vi "filter_edge_detect_3.vi"(0 "image in":T1, 1 "mid Lane Options":T2 {"Edge Polarity" items=["All Edges", "Rising Edges", "Falling Edges"]; "Minimum Edge Strength" format="%.2f"; "Width" step=2; "Kernel Size" step=2}, 2 "right Lane Descriptor":T4, 3 "left Lane Descriptor":T4, 4 "mid Lane Descriptor":T4, 5 "error in (no error)":errorcluster, 6 "Color Plane":i32(ring)=1 items=["Red", "Green", "Blue", "Hue", "Saturation", "Luminance", "Value", "Intensity"], 7 "Lane_center":dbl, 8 "Lane Process":T6(ring)=enum."Get First + Last Edge", 9 "Right Process":T6(ring)=enum."Get First + Last Edge", 10 "Left Options":T2 {"Edge Polarity" items=["All Edges", "Rising Edges", "Falling Edges"]; "Minimum Edge Strength" format="%.2f"; "Width" step=2; "Kernel Size" step=2}, 11 "Right Options":T2 {"Edge Polarity" items=["All Edges", "Rising Edges", "Falling Edges"]; "Minimum Edge Strength" format="%.2f"; "Width" step=2; "Kernel Size" step=2}, 12 "Left Process":T6(ring)=enum."Get First + Last Edge") -> (13 "right_edge_location":cluster{"X":sgl, "Y":sgl}[](array[cluster]), 14 "image out":T1, 15 "Mid Edge Information":T5[](array[typedef]) {"Distance (Real-World)" format="%.2f"; "Location (Real-World)"."Y" format="%.2g"; "Location (Real-World)"."X" format="%.2f"; "Noise" format="%.2f"; "Location (Pixel)"."Y" format="%.2g"; "Location (Pixel)"."X" format="%.2f"; "Strength" format="%.2f"; "Distance (Pixel)" format="%.2f"}, 16 "Left Edge Information":T5[](array[typedef]) {"Distance (Real-World)" format="%.2f"; "Location (Real-World)"."Y" format="%.2g"; "Location (Real-World)"."X" format="%.2f"; "Noise" format="%.2f"; "Location (Pixel)"."Y" format="%.2g"; "Location (Pixel)"."X" format="%.2f"; "Strength" format="%.2f"; "Distance (Pixel)" format="%.2f"}, 17 "Right Edge Information":T5[](array[typedef]) {"Distance (Real-World)" format="%.2f"; "Location (Real-World)"."Y" format="%.2g"; "Location (Real-World)"."X" format="%.2f"; "Noise" format="%.2f"; "Location (Pixel)"."Y" format="%.2g"; "Location (Pixel)"."X" format="%.2f"; "Strength" format="%.2f"; "Distance (Pixel)" format="%.2f"}, 18 "mid_edge_location":cluster{"X":sgl, "Y":sgl}[](array[cluster]), 19 "left_edge_location":cluster{"X":sgl, "Y":sgl}[](array[cluster]))   [LabVIEW 2024]
uses:
  <vilib>/vision/Measure.llb/Edge New.ctl
  <vilib>/vision/Image Controls.llb/IMAQ Image.ctl
  <vilib>/vision/Measure.llb/Edge Options.ctl
  <vilib>/vision/Measure.llb/Edge Polarity.ctl
  <vilib>/vision/NI_Vision_Development_Module.lvlib
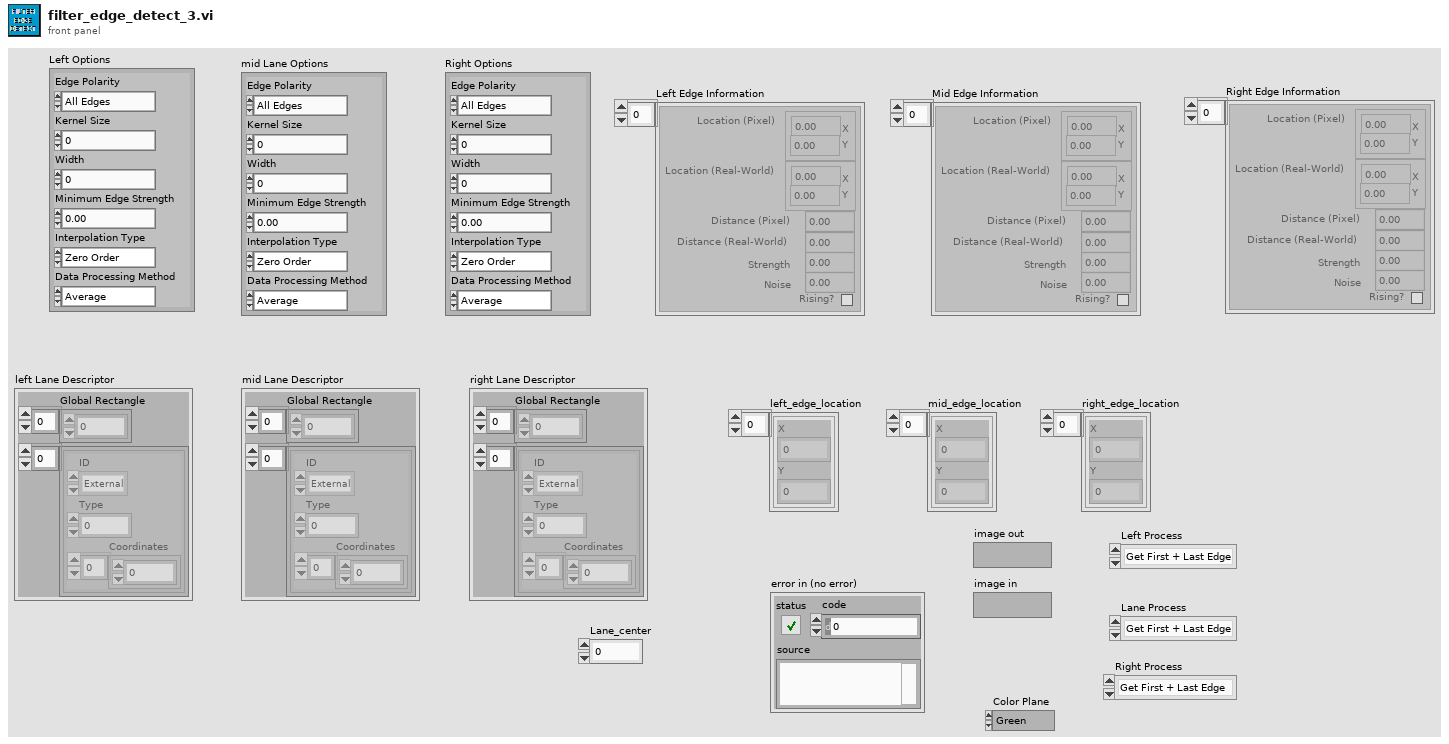
[diagram p1: front panel]
types:
  T1 = typedef "IMAQ Image.ctl" = refnum<image>
  T2 = typedef "Edge Options.ctl" = cluster{"Edge Polarity":T3, "Kernel Size":u32, "Width":u32, "Minimum Edge Strength":sgl, "Interpolation Type":enum32{"Zero Order", "Bilinear", "Quadratic", "Cubic", "Bilinear Fixed"}, "Data Processing Method":enum32{"Average", "Median"}}
  T3 = typedef "Edge Polarity.ctl" = u32
  T4 = cluster{"Global Rectangle":i32[], cluster{"ID":enum32{"External", "Internal"}, "Type":u32, "Coordinates":i32[]}[]}
  T5 = typedef "Edge New.ctl" = cluster{"Location (Pixel)":cluster{"X":sgl, "Y":sgl}, "Location (Real-World)":cluster{"X":sgl, "Y":sgl}, "Distance (Pixel)":dbl, "Distance (Real-World)":dbl, "Strength":dbl, "Noise":dbl, "Rising?":bool}
  T6 = enum16{"Get First Edge", "Get First + Last Edge", "Get All Edges", "Get Best Edge"}
  T7 = cluster{"ID":enum32{"External", "Internal"}, "Type":u32, "Coordinates":i32[]}[]
  T8 = cluster{"ID":enum32{"External", "Internal"}, "Type":u32, "Coordinates":i32[]}
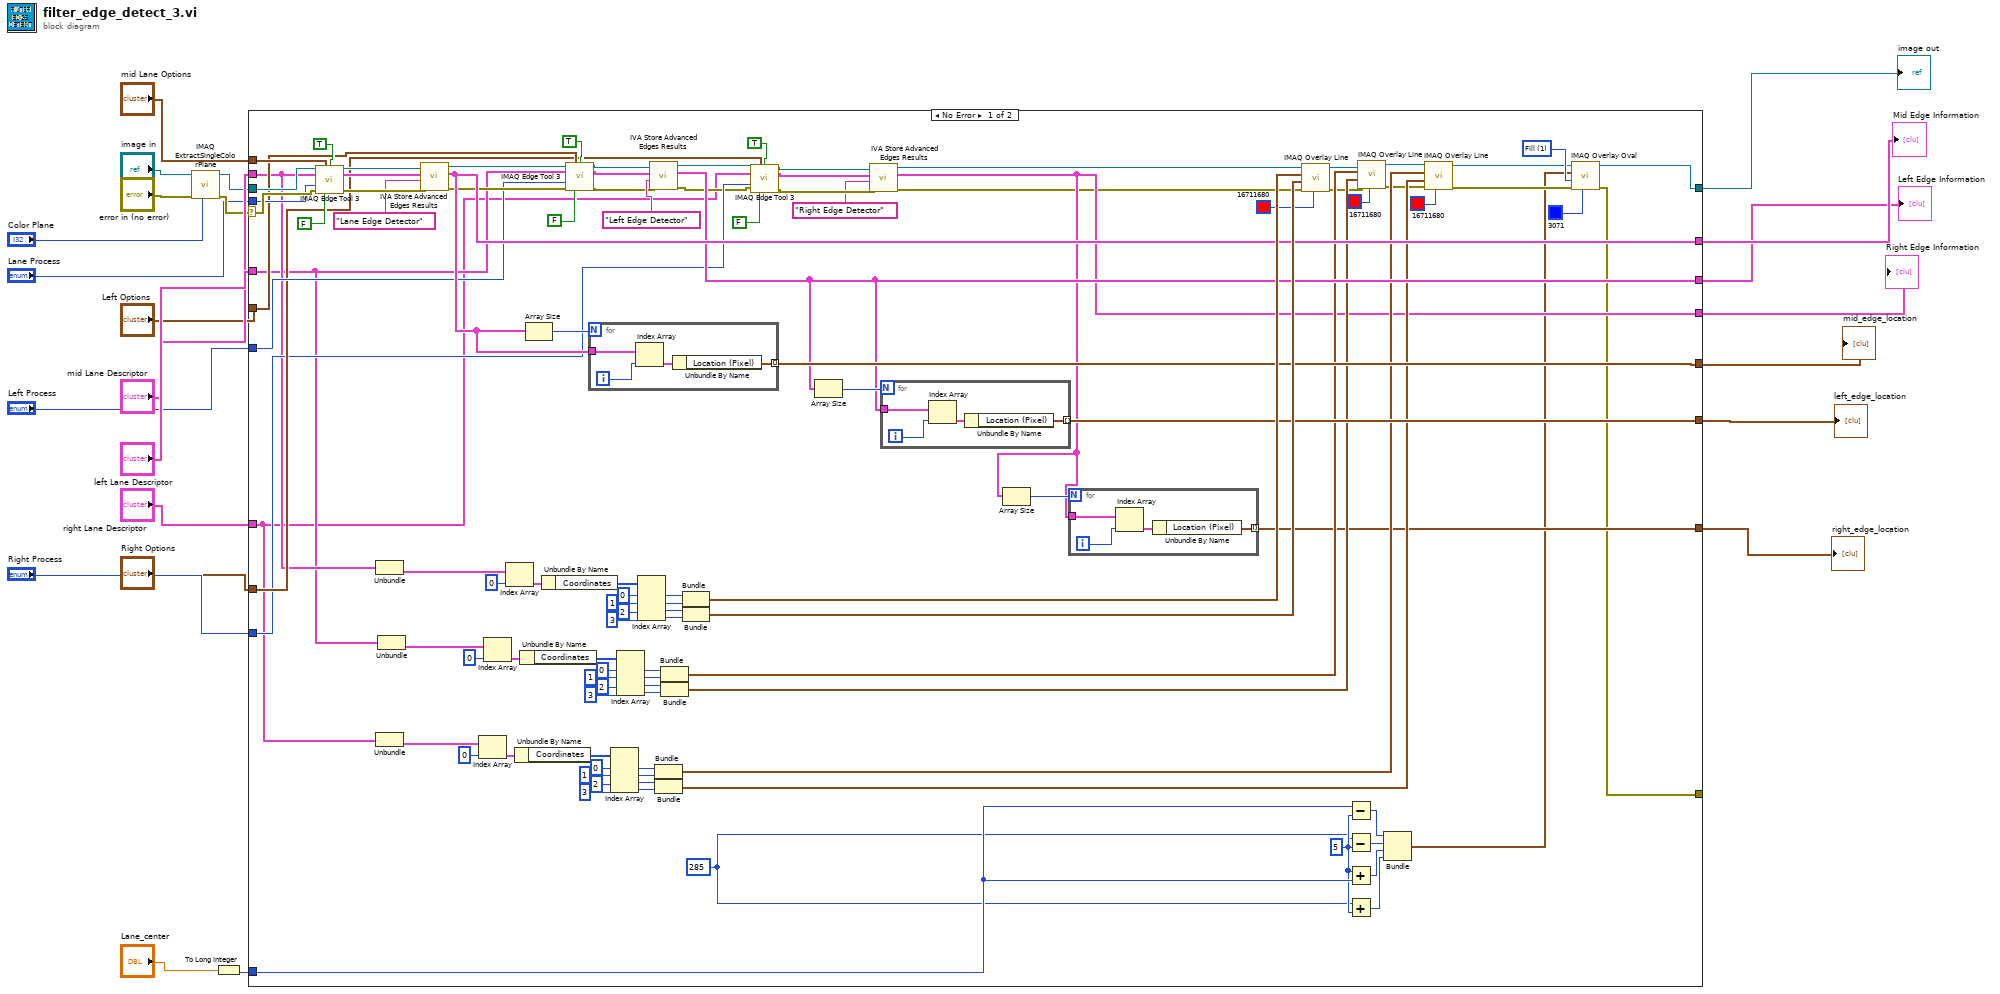
[diagram p0: block diagram]
diagram:
  n1 = call "IMAQ ExtractSingleColorPlane"("Color Plane"="Color Plane", "error in (no error)"="error in (no error)", "Image Src"="image in") -> ("error out"=w4:errorcluster, "Image Dst Out"=w5:T1)  [unwired: 1 in, 6 out]
  n2 = To Long Integer(number="Lane_center") -> (32bit integer=w22:i32)
  n3 = case shown="No Error" w4 {
    selector: w4 -> [w130 w144]
    tunnel: [w33 w144] -> _
    tunnel: w5 -> [w129 w143]
    tunnel: "mid Lane Descriptor" -> [w44 _]
    tunnel: "Lane Process" -> [w128 _]
    tunnel: "mid Lane Options" -> [w126 _]
    tunnel: [w98 _] -> w17
    tunnel: "left Lane Descriptor" -> [w41 _]
    tunnel: "Left Options" -> [w97 _]
    tunnel: "Left Process" -> [w95 _]
    tunnel: [w94 _] -> w19
    tunnel: [w74 _] -> w16
    tunnel: [w75 _] -> w20
    tunnel: "right Lane Descriptor" -> [w39 _]
    tunnel: "Right Options" -> [w69 _]
    tunnel: "Right Process" -> [w68 _]
    tunnel: [w51 _] -> w18
    tunnel: [w35 w143] -> w12
    tunnel: [w38 _] -> w21
    tunnel: w22 -> [w30 _]
    frame No Error {
      w24 = 285 ("y")
      w27 = 5 ("y")
      w37 = u32 1 items=["Frame", "Fill"] ("Drawing Mode (Frame)")
      n4 = call "IMAQ Edge Tool 3"("Image"=w129, "Edge Options"=w126, "Optimized Mode"=TRUE, "ROI Descriptor"=w44, "Process"=w128, "error in (no error)"=w130, "Reverse Direction"=FALSE) -> ("Image (duplicate)"=w125:T1, "Edge Information"=w124:T5[], "error out"=w122:errorcluster)  [unwired: 6 out]
      n5 = Unbundle(w44) -> (w43:T7)  [unwired: 1 out]
      n6 = Unbundle(w39) -> (w40:T7)  [unwired: 1 out]
      n7 = Unbundle(w41) -> (w42:T7)  [unwired: 1 out]
      n8 = call <vilib>:"IVA Store Advanced Edges Results.vi"("error in (no error)"=w122, "Step Name"="Lane Edge Detector", "Edge Information"=w124, "Image in"=w125) -> ("error out"=w96:errorcluster, "Edge Information dup"=w98:T5[], "Image dup"=w100:T1)  [unwired: 5 out]
      n9 = Index Array(array=w40, index=0 ("인덱스")) -> (element=w65:T8)
      n10 = Index Array(array=w42, index=0 ("인덱스")) -> (element=w77:T8)
      n11 = Index Array(array=w43, index=0 ("인덱스")) -> (element=w119:T8)
      n12 = Unbundle By Name(w65) -> ("Coordinates"=w64:i32[])
      n13 = Unbundle By Name(w77) -> ("Coordinates"=w78:i32[])
      n14 = Array Size(array=w98) -> (size(s)=w99:i32)
      n15 = Unbundle By Name(w119) -> ("Coordinates"=w118:i32[])
      n16 = call "IMAQ Edge Tool 3"("Image"=w100, "Edge Options"=w97, "Optimized Mode"=TRUE, "ROI Descriptor"=w41, "Process"=w95, "error in (no error)"=w96, "Reverse Direction"=FALSE) -> ("Image (duplicate)"=w103:T1, "Edge Information"=w102:T5[], "error out"=w101:errorcluster)  [unwired: 6 out]
      n17 = for {
        N: w99 -> [_]
        tunnel: w98 -> [w142]
        tunnel: [w139] -> w94 mode=indexing
        i -> [w141]
        n18 = Index Array(array=w142, index=w141) -> (element=w140:T5)
        n19 = Unbundle By Name(w140) -> ("Location (Pixel)"=w139:cluster{"X":sgl, "Y":sgl})
      }
      n20 = Index Array(array=w64, index #1=0 ("인덱스"), index #2=1 ("인덱스"), index #3=2 ("인덱스"), index #4=3 ("인덱스")) -> (element #1=w59:i32, element #2=w58:i32, element #3=w57:i32, element #4=w56:i32)
      n21 = Index Array(array=w78, index #1=0 ("인덱스"), index #2=1 ("인덱스"), index #3=2 ("인덱스"), index #4=3 ("인덱스")) -> (element #1=w83:i32, element #2=w84:i32, element #3=w85:i32, element #4=w86:i32)
      n22 = Index Array(array=w118, index #1=0 ("인덱스"), index #2=1 ("인덱스"), index #3=2 ("인덱스"), index #4=3 ("인덱스")) -> (element #1=w113:i32, element #2=w112:i32, element #3=w111:i32, element #4=w110:i32)
      n23 = call <vilib>:"IVA Store Advanced Edges Results.vi"("error in (no error)"=w101, "Step Name"="Left Edge Detector", "Edge Information"=w102, "Image in"=w103) -> ("error out"=w67:errorcluster, "Edge Information dup"=w74:T5[], "Image dup"=w70:T1)  [unwired: 5 out]
      n24 = Bundle(w59, w58) -> (w54:cluster{i32, i32})  [unwired: 1 in]
      n25 = Bundle(w57, w56) -> (w53:cluster{i32, i32})  [unwired: 1 in]
      n26 = Bundle(w83, w84) -> (w73:cluster{i32, i32})  [unwired: 1 in]
      n27 = Bundle(w85, w86) -> (w72:cluster{i32, i32})  [unwired: 1 in]
      n28 = Bundle(w113, w112) -> (w109:cluster{i32, i32})  [unwired: 1 in]
      n29 = Bundle(w111, w110) -> (w108:cluster{i32, i32})  [unwired: 1 in]
      n30 = call "IMAQ Edge Tool 3"("Image"=w70, "Edge Options"=w69, "Optimized Mode"=TRUE, "ROI Descriptor"=w39, "Process"=w68, "error in (no error)"=w67, "Reverse Direction"=FALSE) -> ("Image (duplicate)"=w91:T1, "Edge Information"=w92:T5[], "error out"=w93:errorcluster)  [unwired: 6 out]
      n31 = Array Size(array=w74) -> (size(s)=w87:i32)
      n32 = call <vilib>:"IVA Store Advanced Edges Results.vi"("error in (no error)"=w93, "Step Name"="Right Edge Detector", "Edge Information"=w92, "Image in"=w91) -> ("error out"=w47:errorcluster, "Edge Information dup"=w51:T5[], "Image dup"=w50:T1)  [unwired: 5 out]
      n33 = for {
        N: w87 -> [_]
        tunnel: w74 -> [w138]
        tunnel: [w135] -> w75 mode=indexing
        i -> [w137]
        n34 = Index Array(array=w138, index=w137) -> (element=w136:T5)
        n35 = Unbundle By Name(w136) -> ("Location (Pixel)"=w135:cluster{"X":sgl, "Y":sgl})
      }
      n36 = Array Size(array=w51) -> (size(s)=w52:i32)
      n37 = for {
        N: w52 -> [_]
        tunnel: w51 -> [w134]
        tunnel: [w131] -> w38 mode=indexing
        i -> [w133]
        n38 = Index Array(array=w134, index=w133) -> (element=w132:T5)
        n39 = Unbundle By Name(w132) -> ("Location (Pixel)"=w131:cluster{"X":sgl, "Y":sgl})
      }
      n40 = call "IMAQ Overlay Line"("Color"=u32 16711680, "error in (no error)"=w47, "End Point"=w108, "Start Point"=w109, "Image"=w50) -> ("error out"=w46:errorcluster, "Image Out"=w49:T1)  [unwired: 5 in]
      n41 = Subtract(x=w30, y=w27) -> (x-y=w29:i32)
      n42 = Subtract(x=w24, y=w27) -> (x-y=w26:i32)
      n43 = Add(x=w27, y=w30) -> (x+y=w28:i32)
      n44 = Add(x=w24, y=w27) -> (x+y=w25:i32)
      n45 = call "IMAQ Overlay Line"("Color"=u32 16711680, "error in (no error)"=w46, "End Point"=w72, "Start Point"=w73, "Image"=w49) -> ("error out"=w45:errorcluster, "Image Out"=w48:T1)  [unwired: 5 in]
      n46 = Bundle(w29, w26, w28, w25) -> (w32:cluster{i32, i32, i32, i32})  [unwired: 1 in]
      n47 = call "IMAQ Overlay Line"("Color"=u32 16711680, "error in (no error)"=w45, "End Point"=w53, "Start Point"=w54, "Image"=w48) -> ("error out"=w34:errorcluster, "Image Out"=w36:T1)  [unwired: 5 in]
      n48 = call "IMAQ Overlay Oval"("Color"=u32 3071, "error in (no error)"=w34, "Drawing Mode (Frame)"=w37, "Bounding Rectangle"=w32, "Image"=w36) -> ("error out"=w33:errorcluster, "Image Out"=w35:T1)  [unwired: 5 in]
    }
    frame Error {
    }
  }
  "right_edge_location" <- w21
  "left_edge_location" <- w20
  "mid_edge_location" <- w19
  "Right Edge Information" <- w18
  "Mid Edge Information" <- w17
  "Left Edge Information" <- w16
  "image out" <- w12
